vi "Measurement Logic.vi"(8 "error in":errorcluster, 9 "measurement configuration":T2={"Automation Test"=FALSE, "Power sequencing file path"="", "SMU name"="", "SMU channel"="0", "RFSG name"="5842_0", "RFSG port"="", "RFSG attenuation mode"=enum."Constant Attenuation", "RFSG external attenuation (dB)"=2.0, "RFSG s-parameters orientation"=enum."Port2 Towards DUT", "RFSG s2p file path"="", "RFmx name"="5842_0", "RFmx port"="", "RFmx attenuation mode"=enum."Constant Attenuation", "RFmx external attenuation (dB)"=1.2, "RFmx attenuation path name"="", "RFmx s-parameters orientation"=enum."Port2 Towards DUT", "RFmx attenuation s2p path name"="", "RFmx s2p file path"="", "Compression_Expected DUT Gain (dB)"=17.5, "Compression_Max Linear Range (dBm)"=-10.0, "Compression_Compression Point (dB)"=1.0, "Compression_Target Pin (dBm)"=1.0, "Compression_RFSG Frequency Start (Hz)"=10000000000.0, "Compression_RFSG Frequency Stop (Hz)"=18000000000.0, "Compression_RFSG Number of Frequency Step"=10, "Compression_RFSG Power Start (dBm)"=-20.0, "Compression_RFSG Power Stop(dBm)"=1.0, "Compression_RFSG Power Step Size (dB)"=4.0, "Compression_RBW (Hz)"=0.0, "Compression_RF Measurement Interval (s)"=0.0, "Compression_DC Measurement Interval (s)"=0.001, "Compression_Stimulus Mode"=enum."Constant Power and RF", "CP_CW_DC Source Delay (s)"=0.0, "CP_PRF_DC Source Delay (s)"=0.0, "CP_PRF_RFmx Trigger Delay (s)"=0.0, "CP_PRF_RF Pulse Width (s)"=0.0001, "CP_PRF_PRI (s)"=0.001, "PP_PRF_DC Source Delay (s)"=0.0, "PP_PRF_RFmx Trigger Delay (s)"=0.0, "PP_PRF_RF Pulse Width (s)"=0.0001, "PP_PRF_PRI (s)"=0.001, "PP_PRF_DC Pulse Width (s)"=0.0008, "PP_PRF_ON Current Limit (A)"=2.0, "PP_PRF_Bias Voltage Level (V)"=0.0, "PP_PRF_Bias Current Limit (A)"=0.2, "Power sequencing file validity check"=FALSE} {"Compression_Target Pin (dBm)" format="%#pdBm"; "PP_PRF_Bias Current Limit (A)" format="%#pA"; "PP_PRF_Bias Voltage Level (V)" format="%#pV"; "PP_PRF_ON Current Limit (A)" format="%#pA"; "PP_PRF_DC Pulse Width (s)" format="%#ps"; "PP_PRF_PRI (s)" format="%#ps"; "PP_PRF_RF Pulse Width (s)" format="%#ps"; "PP_PRF_RFmx Trigger Delay (s)" format="%#ps"; "PP_PRF_DC Source Delay (s)" format="%#ps"; "CP_PRF_PRI (s)" format="%#ps"; "CP_PRF_RF Pulse Width (s)" format="%#ps"; "CP_PRF_RFmx Trigger Delay (s)" format="%#ps"; "CP_PRF_DC Source Delay (s)" format="%#ps"; "CP_CW_DC Source Delay (s)" format="%#ps"; "Compression_DC Measurement Interval (s)" format="%#ps"; "Compression_RF Measurement Interval (s)" format="%#ps"; "RFmx external attenuation (dB)" format="%.2f"; "RFSG external attenuation (dB)" format="%.2f"}, 10 "measure call context in":refnum<class "Measure Call Context.lvclass">) -> (0 "error out":errorcluster, 1 "measurement results":T1, 2 "measure call context out":refnum<class "Measure Call Context.lvclass">)   [LabVIEW 2023, in "FPT_Compression.lvclass"]
doc: "Contains the core logic for executing the measurement."
uses:
  FPT_Compression.lvclass
  <vilib>/Plug-In SDKs/Measurements/Measure Call Context/Measure Call Context.lvclass
  Measurement Configuration.ctl
  Measurement Results.ctl
  <vilib>/Analysis/baseanly.llb/Mean (DBL).vi
  <extravilib>/ChannelInstances/Event Messenger-bool/Instantiate.vi
  <vilib>/Analysis/NI_AALBase.lvlib
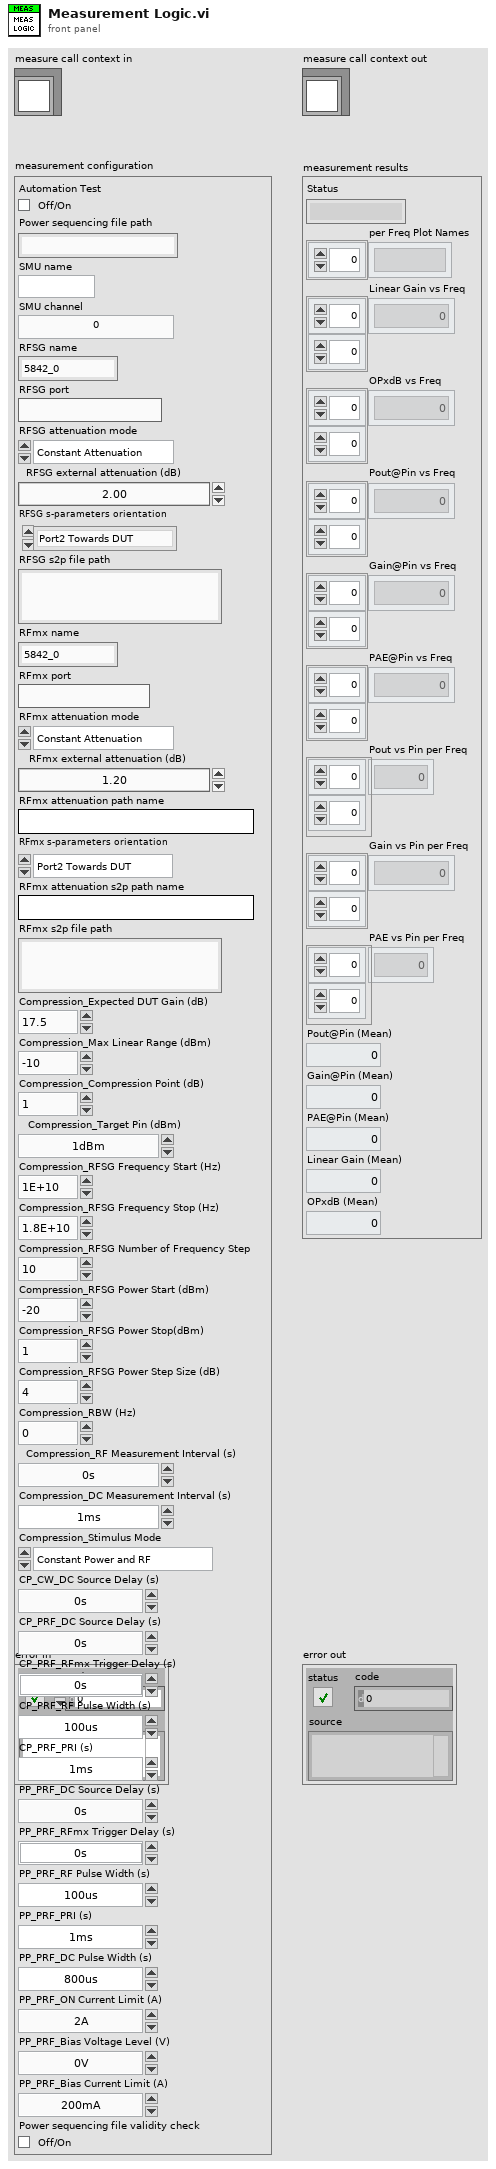
[diagram p1: front panel]
types:
  T1 = typedef "FPT_Compression.lvclass/Measurement Results.ctl" = cluster{"Status":string, "per Freq Plot Names":string[], "Linear Gain vs Freq":dbl[][], "OPxdB vs Freq":dbl[][], "Pout@Pin vs Freq":dbl[][], "Gain@Pin vs Freq":dbl[][], "PAE@Pin vs Freq":dbl[][], "Pout vs Pin per Freq":dbl[][], "Gain vs Pin per Freq":dbl[][], "PAE vs Pin per Freq":dbl[][], "Pout@Pin (Mean)":dbl, "Gain@Pin (Mean)":dbl, "PAE@Pin (Mean)":dbl, "Linear Gain (Mean)":dbl, "OPxdB (Mean)":dbl}
  T2 = typedef "FPT_Compression.lvclass/Measurement Configuration.ctl" = cluster{"Automation Test":bool, "Power sequencing file path":string, "SMU name":string, "SMU channel":string, "RFSG name":string, "RFSG port":string, "RFSG attenuation mode":enum32{"<None>", "Constant Attenuation", "s2p File"}, "RFSG external attenuation (dB)":dbl, "RFSG s-parameters orientation":enum32{"Port1 Towards DUT", "Port2 Towards DUT"}, "RFSG s2p file path":string, "RFmx name":string, "RFmx port":string, "RFmx attenuation mode":enum32{"<None>", "Constant Attenuation", "s2p File"}, "RFmx external attenuation (dB)":dbl, "RFmx attenuation path name":string, "RFmx s-parameters orientation":enum32{"Port1 Towards DUT", "Port2 Towards DUT"}, "RFmx attenuation s2p path name":string, "RFmx s2p file path":string, "Compression_Expected DUT Gain (dB)":dbl, "Compression_Max Linear Range (dBm)":dbl, "Compression_Compression Point (dB)":dbl, "Compression_Target Pin (dBm)":dbl, "Compression_RFSG Frequency Start (Hz)":dbl, "Compression_RFSG Frequency Stop (Hz)":dbl, "Compression_RFSG Number of Frequency Step":i32, "Compression_RFSG Power Start (dBm)":dbl, "Compression_RFSG Power Stop(dBm)":dbl, "Compression_RFSG Power Step Size (dB)":dbl, "Compression_RBW (Hz)":dbl, "Compression_RF Measurement Interval (s)":dbl, "Compression_DC Measurement Interval (s)":dbl, "Compression_Stimulus Mode":enum32{"Constant Power and RF", "Constant Power and Pulsed RF", "Pulsed Power and RF"}, "CP_CW_DC Source Delay (s)":dbl, "CP_PRF_DC Source Delay (s)":dbl, "CP_PRF_RFmx Trigger Delay (s)":dbl, "CP_PRF_RF Pulse Width (s)":dbl, "CP_PRF_PRI (s)":dbl, "PP_PRF_DC Source Delay (s)":dbl, "PP_PRF_RFmx Trigger Delay (s)":dbl, "PP_PRF_RF Pulse Width (s)":dbl, "PP_PRF_PRI (s)":dbl, "PP_PRF_DC Pulse Width (s)":dbl, "PP_PRF_ON Current Limit (A)":dbl, "PP_PRF_Bias Voltage Level (V)":dbl, "PP_PRF_Bias Current Limit (A)":dbl, "Power sequencing file validity check":bool}
  T3 = enum32{"Power On Dut", "De-embedding + Measurement", "Power Off Dut"}[]
  T4 = cluster{"measurement configuration":T2, "measurement results":T1, "CustomData":cluster{"Valid CSV":bool}}
  T5 = typedef "RFmx Config - Compression.ctl" = cluster{"RFmx Name":refnum<k15>, "RFmx Port":string, "Attenuation":cluster{"Mode":enum32{"<None>", "Constant Attenuation", "s2p File"}, "Constant Attenuation":cluster{"RFmx External Attenuation (dB)":dbl}, "s2p File":cluster{"RFmx S-Parameters Orientation":i32, "RFmx Attenuation s2p File":path}}}
  T6 = typedef "RFSG Config - Compression.ctl" = cluster{"RFSG Name":refnum<k15>, "RFSG Port":string, "Attenuation":cluster{"Mode":enum32{"<None>", "Constant Attenuation", "s2p File"}, "Contant Attenuation":cluster{"RFSG External Attenuation (dB)":dbl}, "s2p File":cluster{"RFSG S-parameters Orientation":i32, "RFSG s2p File Path":path}}}
  T7 = typedef "Test Config - Compression.ctl" = cluster{"Expected DUT Gain (dB)":dbl, "Max Linear Range (dBm)":dbl, "Compression Point (dB)":dbl, "Pout at Pin (dBm)":dbl, "RFSG Frequency Start (Hz)":dbl, "RFSG Frequency Stop (Hz)":dbl, "RFSG Number of Frequency Step":i32, "Power Start (dBm)":dbl, "Power Stop(dBm)":dbl, "Power Step Size (dB)":dbl, "RBW (Hz)":dbl, "Modes":cluster{"RF Measurement Interval (s)":dbl, "DC Measurement Interval (s)":dbl, "Power Stimulus Mode":enum16{"Constant Power and RF", "Constant Power and Pulsed RF", "Pulsed Power and RF"}, "CP_CW_DC Source Delay (s)":dbl, "CP_PRF_DC Source Delay (s)":dbl, "CP_PRF_RFmx Trigger Delay (s)":dbl, "CP_PRF_RF Pulse Width (s)":dbl, "CP_PRF_PRI (s)":dbl, "PP_PRF_DC Source Delay (s)":dbl, "PP_PRF_RFmx Trigger Delay (s)":dbl, "PP_PRF_RF Pulse Width (s)":dbl, "PP_PRF_PRI (s)":dbl, "PP_PRF_DC Pulse Width (s)":dbl, "PP_PRF_Bias Voltage Level (V)":dbl, "PP_PRF_Bias Current Limit (A)":dbl}}
  T8 = typedef "SMU Config - Compression.ctl" = cluster{"SMU Name":refnum<k15>, "SMU Channel":string, "IDD Current Limit (A)":dbl}
  T9 = typedef "Results - Compression.ctl" = cluster{"Linear Gain vs Freq":dbl[][], "OPxdb vs Freq":dbl[][], "Pout@Pin vs Freq":dbl[][], "Gain@Pin vs Freq":dbl[][], "PAE@Pin vs Freq":dbl[][], "Pout vs Pin per Freq":dbl[][], "Gain vs Pin per Freq":dbl[][], "PAE vs Pin per Freq":dbl[][]}
  T10 = typedef "Event Messenger-bool.lvlib/))Channel.ctl" = refnum<queue>
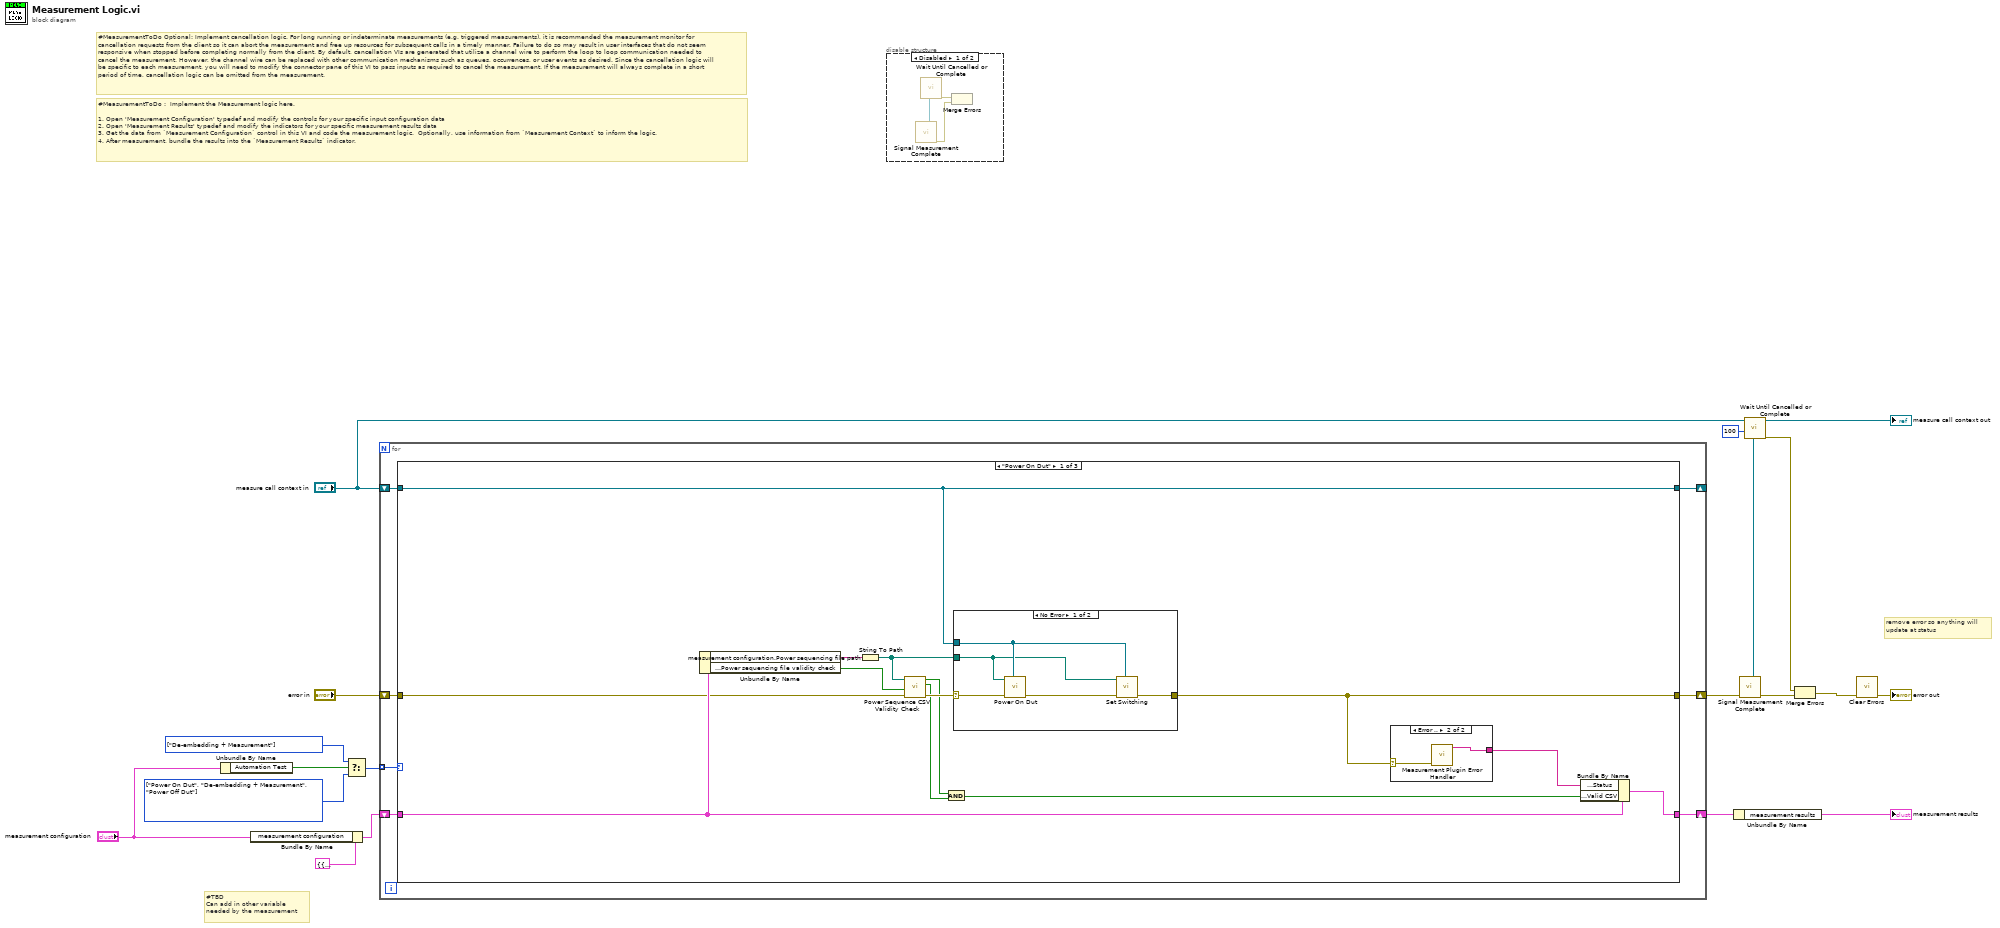
[diagram p0: block diagram]
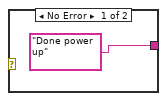
[diagram p3: hidden frame]
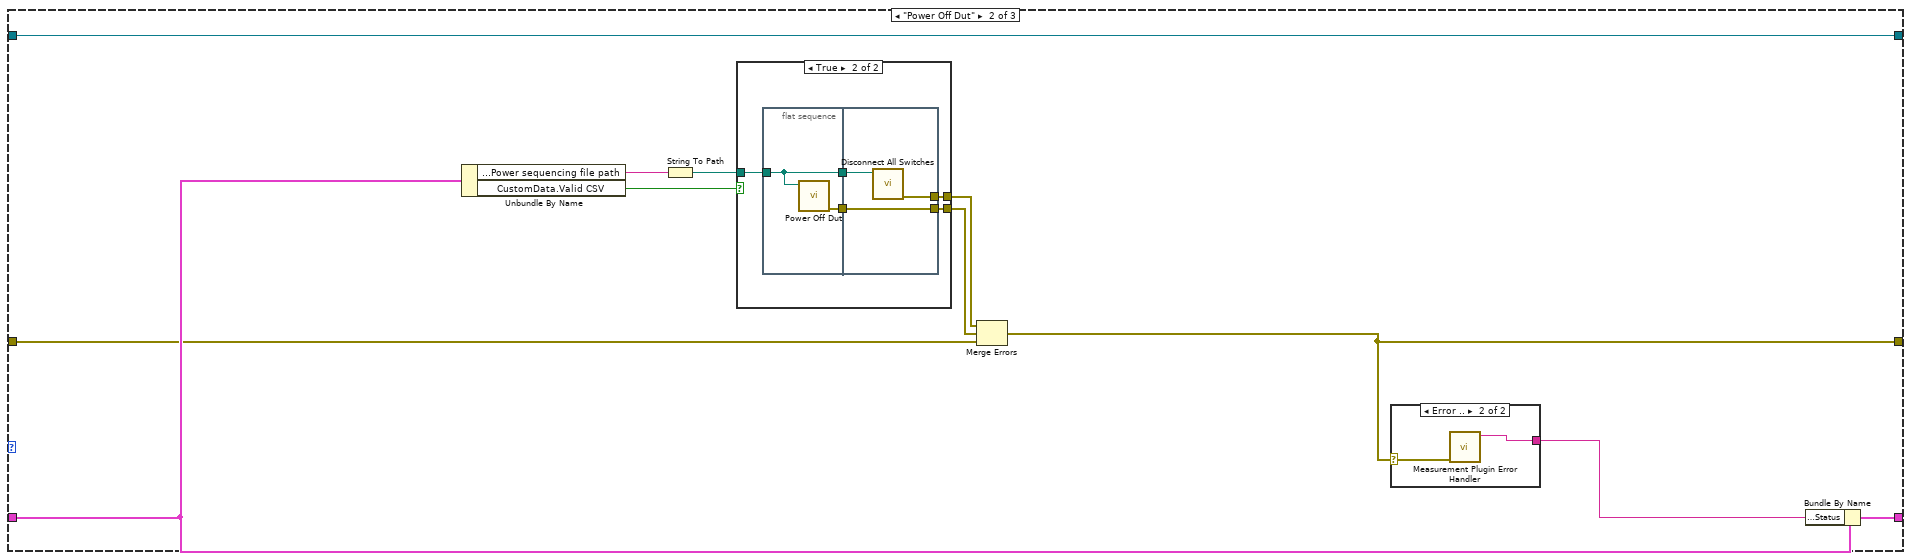
[diagram p4: hidden frame]
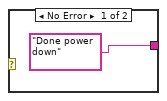
[diagram p6: hidden frame]
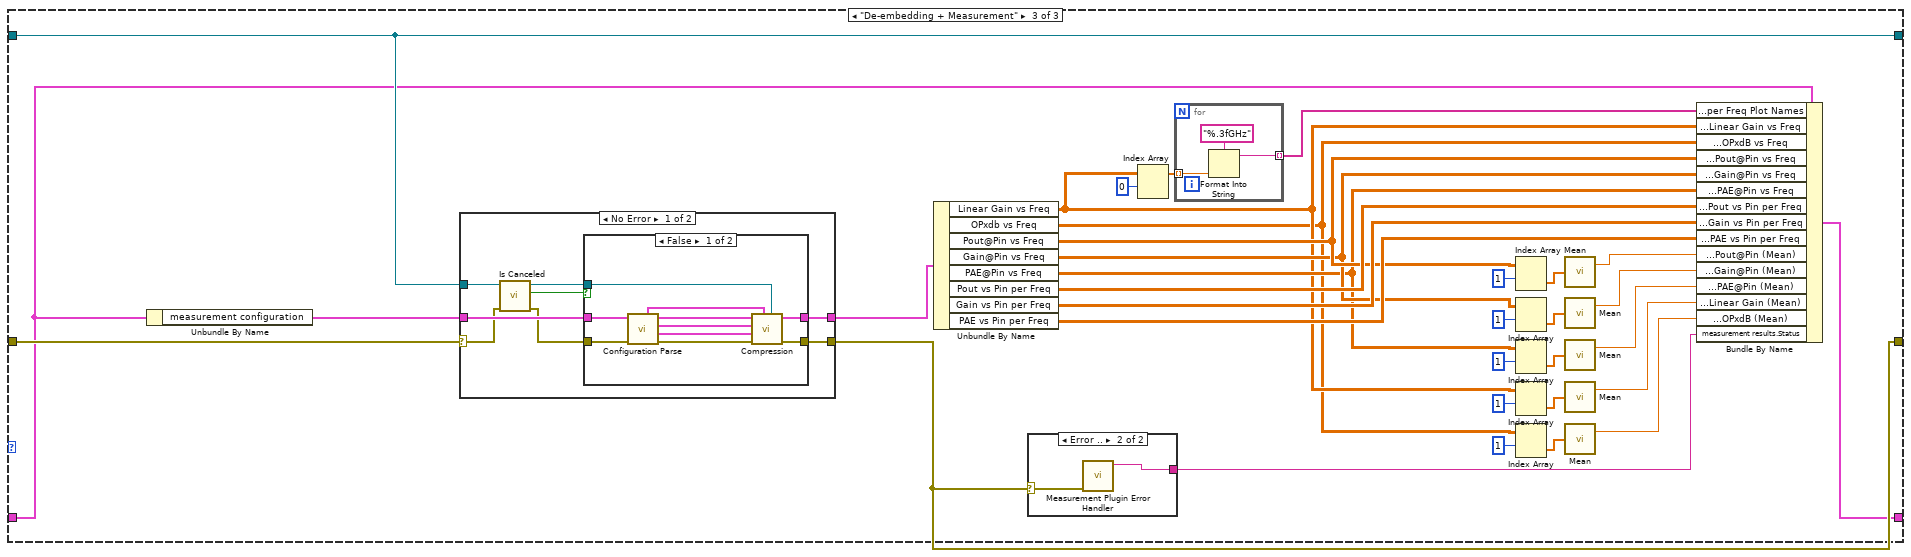
[diagram p7: hidden frame]
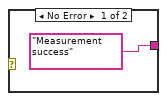
[diagram p10: hidden frame]
diagram:
  w12 = T3 [enum."De-embedding + Measurement"] items=["Power On Dut", "De-embedding + Measurement", "Power Off Dut"]
  w14 = T3 [enum."Power On Dut", enum."De-embedding + Measurement", enum."Power Off Dut"] items=["Power On Dut", "De-embedding + Measurement", "Power Off Dut"]
  # "remove error so anything will\nupdate at status"
  # "#TBD\nCan add in other variable\nneeded by the measurement"
  # "#MeasurementToDo Optional: Implement cancellation logic. For long running or indeterminate measurements (e.g. triggered measurements), it is recommended the measurement monitor for cancellation requests from the client so it can abort the measurement and free up resources for subsequent calls in a timely manner. Failure to do so may result in user interfaces that do not seem responsive when stopped before completing normally from the client. By default, cancellation VIs are generated that utilize a channel wire to perform the loop to loop communication needed to cancel the measurement. However, the channel wire can be replaced with other communication mechanisms such as queues, occurrences, or user events as desired. Since the cancellation logic will be specific to each measurement, you will need to modify the connector pane of this VI to pass inputs as required to cancel the measurement. If the measurement will always complete in a short period of time, cancellation logic can be omitted from the measurement."
  # "#MeasurementToDo :  Implement the Measurement logic here.\n\n1. Open 'Measurement Configuration' typedef and modify the controls for your specific input configuration data\n2. Open 'Measurement Results' typedef and modify the indicators for your specific measurement results data\n3. Get the data from `Measurement Configuration` control in this VI and code the measurement logic.  Optionally, use information from `Measurement Context` to inform the logic.\n4. After measurement, bundle the results into the `Measurement Results` indicator."
  n1 = Unbundle By Name("measurement configuration") -> ("Automation Test"=w10:bool)
  n2 = Bundle By Name(cluster=T4 {"measurement configuration"={"Automation Test"=FALSE, "Power sequencing file path"="", "SMU name"="", "SMU channel"="0", "RFSG name"="5842_0", "RFSG port"="", "RFSG attenuation mode"=enum."Constant Attenuation", "RFSG external attenuation (dB)"=2.0, "RFSG s-parameters orientation"=enum."Port2 Towards DUT", "RFSG s2p file path"="", "RFmx name"="5842_0", "RFmx port"="", "RFmx attenuation mode"=enum."Constant Attenuation", "RFmx external attenuation (dB)"=1.2, "RFmx attenuation path name"="", "RFmx s-parameters orientation"=enum."Port2 Towards DUT", "RFmx attenuation s2p path name"="", "RFmx s2p file path"="", "Compression_Expected DUT Gain (dB)"=17.5, "Compression_Max Linear Range (dBm)"=-10.0, "Compression_Compression Point (dB)"=1.0, "Compression_Target Pin (dBm)"=1.0, "Compression_RFSG Frequency Start (Hz)"=10000000000.0, "Compression_RFSG Frequency Stop (Hz)"=18000000000.0, "Compression_RFSG Number of Frequency Step"=10, "Compression_RFSG Power Start (dBm)"=-20.0, "Compression_RFSG Power Stop(dBm)"=1.0, "Compression_RFSG Power Step Size (dB)"=4.0, "Compression_RBW (Hz)"=0.0, "Compression_RF Measurement Interval (s)"=0.0, "Compression_DC Measurement Interval (s)"=0.001, "Compression_Stimulus Mode"=enum."Constant Power and RF", "CP_CW_DC Source Delay (s)"=0.0, "CP_PRF_DC Source Delay (s)"=0.0, "CP_PRF_RFmx Trigger Delay (s)"=0.0, "CP_PRF_RF Pulse Width (s)"=0.0001, "CP_PRF_PRI (s)"=0.001, "PP_PRF_DC Source Delay (s)"=0.0, "PP_PRF_RFmx Trigger Delay (s)"=0.0, "PP_PRF_RF Pulse Width (s)"=0.0001, "PP_PRF_PRI (s)"=0.001, "PP_PRF_DC Pulse Width (s)"=0.0008, "PP_PRF_ON Current Limit (A)"=2.0, "PP_PRF_Bias Voltage Level (V)"=0.0, "PP_PRF_Bias Current Limit (A)"=0.2, "Power sequencing file validity check"=FALSE}, "measurement results"={"Status"="", "per Freq Plot Names"=[], "Linear Gain vs Freq"=[], "OPxdB vs Freq"=[], "Pout@Pin vs Freq"=[], "Gain@Pin vs Freq"=[], "PAE@Pin vs Freq"=[], "Pout vs Pin per Freq"=[], "Gain vs Pin per Freq"=[], "PAE vs Pin per Freq"=[], "Pout@Pin (Mean)"=0.0, "Gain@Pin (Mean)"=0.0, "PAE@Pin (Mean)"=0.0, "Linear Gain (Mean)"=0.0, "OPxdB (Mean)"=0.0}, "CustomData"={"Valid CSV"=FALSE}}, "measurement configuration"="measurement configuration") -> (w18:T4)
  n3 = Select(t=w12, s=w10, f=w14) -> (s? t:f=w13:T3)
  n4 = for {
    tunnel: w13 -> [w25] mode=indexing
    shift-right: [w20] -> w8
    shift-left: "error in" -> [w26]
    shift-right: [w21] -> w17
    shift-left: w18 -> [w24]
    shift-right: [w22] -> _
    shift-left: "measure call context in" -> [w23]
    n5 = case shown="\"Power On Dut\"" w25 {
      tunnel: w26 -> [w33 w50 w75]
      tunnel: w24 -> [w39 w56 w74]
      tunnel: w23 -> [w34 w54 w104]
      tunnel: [w35 w55 w106] -> w20
      tunnel: [w34 w54 w104] -> w22
      tunnel: [w37 w57 w105] -> w21
      frame "Power On Dut" {
        n6 = Unbundle By Name(w39) -> ("measurement configuration.Power sequencing file path"=w36:string, "measurement configuration.Power sequencing file validity check"=w30:bool)
        n7 = String To Path(string=w36) -> (path=w32:path)
        n8 = call "Power Sequence CSV Validity Check.vi"("error in"=w33, "Enable Validity Check?"=w30, "File Path"=w32) -> ("error out"=w31:errorcluster, "Valid Execution Order"=w28:bool, "All Instruments Available"=w29:bool)  [unwired: 5 in, 1 out]
        n9 = And(x=w29, y=w28) -> (x .and. y?=w27:bool)
        n10 = case shown="No Error" w31 {
          selector: w31 -> [w40 w45]
          tunnel: [w43 w45] -> w35
          tunnel: w34 -> [w42 _]
          tunnel: w32 -> [w41 _]
          frame No Error {
            n11 = call "Power On Dut.vi"("measure call context in"=w42, "error in"=w40, "Power sequencing file path"=w41) -> ("error out"=w44:errorcluster)  [unwired: 7 in, 1 out]
            n12 = call "Set Switching.vi"("measure call context in"=w42, "error in"=w44, "File Path"=w41) -> ("error out"=w43:errorcluster)  [unwired: 7 in, 1 out]
          }
          frame Error {
          }
        }
        n13 = case shown="Error .." w35 {
          selector: w35 -> [_ w48]
          tunnel: ["Done power up" w47] -> w38
          frame No Error {
          }
          frame Error {
            n14 = call "Measurement Plugin Error Handler.vi"("error in"=w48) -> ("Status Message (Error)"=w47:string)  [unwired: 9 in, 1 out]
          }
        }
        n15 = Bundle By Name(cluster=w39, "measurement results.Status"=w38, "CustomData.Valid CSV"=w27) -> (w37:T4)
      }
      frame "Power Off Dut" {
        n16 = Unbundle By Name(w56) -> ("measurement configuration.Power sequencing file path"=w59:string, "CustomData.Valid CSV"=w49:bool)
        n17 = String To Path(string=w59) -> (path=w51:path)
        n18 = case shown="True" w49 {
          tunnel: [_ w62] -> w53
          tunnel: [_ w61] -> w52
          tunnel: w51 -> [_ w60]
          frame False {
            # "Skip if CSV not valid"
          }
          frame True {
            n19 = flat-sequence {
              tunnel: w60 -> [w65]
              tunnel: [w66] -> w64
              tunnel: [w65] -> w63
              tunnel: w64 -> [w69]
              tunnel: w63 -> [w67]
              tunnel: [w69] -> w61
              tunnel: [w68] -> w62
              frame #0 {
                n20 = call "Power Off Dut.vi"("Power Sequencing File Path"=w65) -> ("error out"=w66:errorcluster)  [unwired: 10 in]
              }
              frame #1 {
                n21 = call "Disconnect All Switches.vi"("File Path"=w67) -> ("error out"=w68:errorcluster)  [unwired: 10 in]
              }
            }
          }
        }
        n22 = Merge Errors(w53, w52, w50) -> (w55:errorcluster)
        n23 = case shown="Error .." w55 {
          selector: w55 -> [_ w72]
          tunnel: ["Done power down" w71] -> w58
          frame No Error {
          }
          frame Error {
            n24 = call "Measurement Plugin Error Handler.vi"("error in"=w72) -> ("Status Message (Error)"=w71:string)  [unwired: 9 in, 1 out]
          }
        }
        n25 = Bundle By Name(cluster=w56, "measurement results.Status"=w58) -> (w57:T4)
      }
      frame "De-embedding + Measurement" {
        n26 = Unbundle By Name(w74) -> ("measurement configuration"=w73:T2)
        n27 = case shown="No Error" w75 {
          selector: w75 -> [w108 w126]
          tunnel: [w114 w126] -> w106
          tunnel: w104 -> [w110 _]
          tunnel: [w113 _] -> w96
          tunnel: w73 -> [w112 _]
          frame No Error {
            n28 = call <vilib>:"Is Canceled.vi"("error in"=w108, "measure call context in"=w110) -> ("error out"=w107:errorcluster, "is canceled?"=w111:bool, "measure call context out"=w109:refnum<class "Measure Call Context.lvclass">)  [unwired: 7 in]
            n29 = case shown="False" w111 {
              tunnel: [w124 w125] -> w114
              tunnel: w109 -> [w123 _]
              tunnel: [w122 _] -> w113
              tunnel: w112 -> [w115 _]
              tunnel: w107 -> [w121 w125]
              frame False {
                n30 = call "Configuration Parse.vi"("error in"=w121, "Measurement Configuration"=w115) -> ("error out"=w117:errorcluster, "RFmx Settings"=w118:T5, "RFSG Settings"=w119:T6, "Test Configuration"=w120:T7, "SMU Settings"=w116:T8)  [unwired: 5 in]
                n31 = call "Compression.vi"("measure call context in"=w123, "SMU Settings"=w116, "error in"=w117, "RFmx Settings"=w118, "RFSG Settings"=w119, "Test Configuration"=w120) -> ("error out"=w124:errorcluster, "Data"=w122:T9)  [unwired: 4 in]
              }
              frame True {
                # "Canceled"
              }
            }
          }
          frame Error {
          }
        }
        n32 = Unbundle By Name(w96) -> ("Linear Gain vs Freq"=w82:dbl[][], "OPxdb vs Freq"=w79:dbl[][], "Pout@Pin vs Freq"=w88:dbl[][], "Gain@Pin vs Freq"=w87:dbl[][], "PAE@Pin vs Freq"=w86:dbl[][], "Pout vs Pin per Freq"=w95:dbl[][], "Gain vs Pin per Freq"=w94:dbl[][], "PAE vs Pin per Freq"=w93:dbl[][])
        n33 = case shown="Error .." w106 {
          selector: w106 -> [_ w129]
          tunnel: ["Measurement success" w128] -> w76
          frame No Error {
          }
          frame Error {
            n34 = call "Measurement Plugin Error Handler.vi"("error in"=w129) -> ("Status Message (Error)"=w128:string)  [unwired: 9 in, 1 out]
          }
        }
        n35 = Index Array(array=w82, index (row)=0) -> (element=w100:dbl[])  [unwired: 1 in]
        n36 = for {
          tunnel: w100 -> [w130] mode=indexing
          tunnel: [w131] -> w98 mode=indexing
          # "Get Plot Names"
          n37 = Format Into String(format string="%.3fGHz", w130) -> (resulting string=w131:string)  [unwired: 2 in, 1 out]
        }
        n38 = Index Array(array=w88, index (row)=1) -> (element=w92:dbl[])  [unwired: 1 in]
        n39 = Index Array(array=w87, index (row)=1) -> (element=w89:dbl[])  [unwired: 1 in]
        n40 = Index Array(array=w86, index (row)=1) -> (element=w91:dbl[])  [unwired: 1 in]
        n41 = Index Array(array=w82, index (row)=1) -> (element=w90:dbl[])  [unwired: 1 in]
        n42 = Index Array(array=w79, index (row)=1) -> (element=w81:dbl[])  [unwired: 1 in]
        n43 = call-poly <vilib>:"Mean.vi"("X"=w92) -> ("mean"=w85:dbl)  [unwired: 1 out]
        n44 = call-poly <vilib>:"Mean.vi"("X"=w89) -> ("mean"=w84:dbl)  [unwired: 1 out]
        n45 = call-poly <vilib>:"Mean.vi"("X"=w91) -> ("mean"=w83:dbl)  [unwired: 1 out]
        n46 = call-poly <vilib>:"Mean.vi"("X"=w90) -> ("mean"=w78:dbl)  [unwired: 1 out]
        n47 = call-poly <vilib>:"Mean.vi"("X"=w81) -> ("mean"=w77:dbl)  [unwired: 1 out]
        n48 = Bundle By Name(cluster=w74, "measurement results.per Freq Plot Names"=w98, "measurement results.Linear Gain vs Freq"=w82, "measurement results.OPxdB vs Freq"=w79, "measurement results.Pout@Pin vs Freq"=w88, "measurement results.Gain@Pin vs Freq"=w87, "measurement results.PAE@Pin vs Freq"=w86, "measurement results.Pout vs Pin per Freq"=w95, "measurement results.Gain vs Pin per Freq"=w94, "measurement results.PAE vs Pin per Freq"=w93, "measurement results.Pout@Pin (Mean)"=w85, "measurement results.Gain@Pin (Mean)"=w84, "measurement results.PAE@Pin (Mean)"=w83, "measurement results.Linear Gain (Mean)"=w78, "measurement results.OPxdB (Mean)"=w77, "measurement results.Status"=w76) -> (w105:T4)
      }
    }
  }
  n49 = disable-structure shown="Disabled" {
    frame Disabled {
      n50 = call "Signal Measurement Complete.vi"() -> ("error out"=w134:errorcluster, "done channel"=w135:T10)  [unwired: 10 in]
      n51 = call "Wait Until Cancelled or Complete.vi"("done channel"=w135) -> ("error out"=w133:errorcluster)  [unwired: 9 in, 1 out]
      n52 = Merge Errors(w133, w134) -> ()  [unwired: 1 out]
    }
    frame Enabled {
    }
  }
  n53 = Unbundle By Name(w17) -> ("measurement results"=→"measurement results":T1)
  n54 = call "Signal Measurement Complete.vi"("error in (no error)"=w8) -> ("error out"=w7:errorcluster, "done channel"=w6:T10)  [unwired: 9 in]
  n55 = call "Wait Until Cancelled or Complete.vi"("done channel"=w6, "ms polling interval"=100, "measure call context in"="measure call context in") -> ("error out"=w2:errorcluster, "measure call context out"=→"measure call context out":refnum<class "Measure Call Context.lvclass">)  [unwired: 7 in]
  n56 = Merge Errors(w2, w7) -> (w4:errorcluster)
  n57 = call <vilib>:"Clear Errors.vi"("error in (no error)"=w4) -> ("error out"=→"error out":errorcluster)  [unwired: 5 in, 1 out]
